vi "OFDM_TransimitPreparation.vi"(10 "IQ rate":dbl, 11 "array":cdb[](array[numeric])) -> (3 "output cluster":cluster{"t0":dbl, "dt":dbl, "Y":cdb[]})   [LabVIEW 2022 SP3]
uses:
  <vilib>/Analysis/baseanly.llb/Mean (DBL).vi
  <vilib>/Analysis/NI_AALBase.lvlib
panel:
  out "max index(es)":i32
  out "max value":dbl
  out "Average Power":dbl format="%0.6f"
  out "size(s)":i32
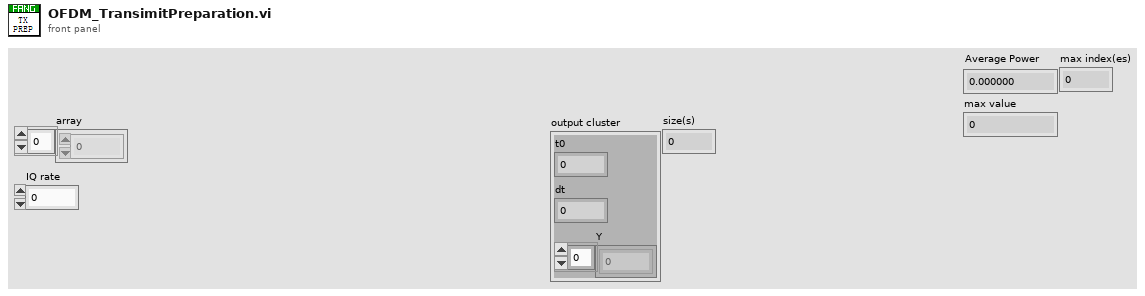
[diagram p1: front panel]
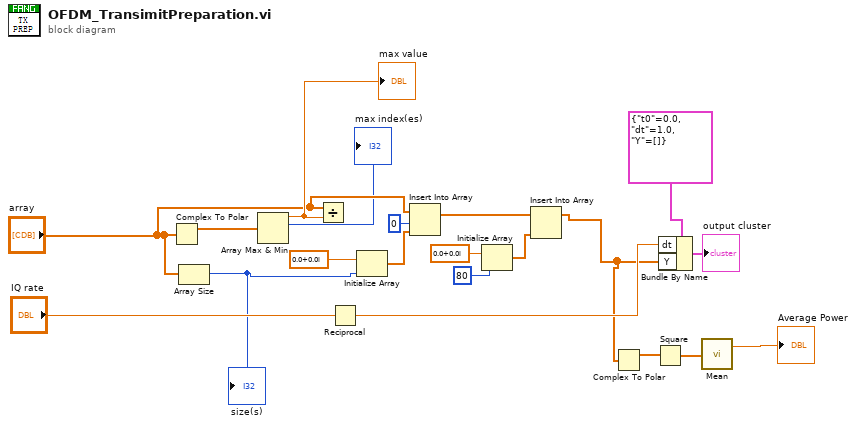
[diagram p0: block diagram]
diagram:
  n1 = Complex To Polar(r * e^(i*theta)="array") -> (r=w20:dbl[])  [unwired: 1 out]
  n2 = Array Size(array="array") -> (size(s)=w7:i32)
  "size(s)" <- w7
  n3 = Array Max & Min(array=w20) -> (max value=w19:dbl, max index (indices)=→"max index(es)":i32)  [unwired: 2 out]
  "max value" <- w19
  n4 = Divide(x="array", y=w19) -> ()  [unwired: 1 out]
  n5 = Reciprocal(x="IQ rate") -> (1/x=w9:dbl)
  n6 = Initialize Array(cdb 0.0+0.0i ("element"), w7) -> (w15:cdb[])
  n7 = Insert Into Array(array="array", index=0, new element=w15) -> (w16:cdb[])
  n8 = Initialize Array(cdb 0.0+0.0i ("element"), 80 ("dimension size")) -> (w14:cdb[])
  n9 = Insert Into Array(array=w16, new element=w14) -> (w3:cdb[])  [unwired: 1 in]
  n10 = Complex To Polar(r * e^(i*theta)=w3) -> (r=w6:dbl[])  [unwired: 1 out]
  n11 = Square(x=w6) -> (x^2=w5:dbl[])
  n12 = Bundle By Name(cluster=cluster{"t0":dbl, "dt":dbl, "Y":cdb[]} {"t0"=0.0, "dt"=1.0, "Y"=[]} ("data"), "dt"=w9, "Y"=w3) -> (→"output cluster":cluster{"t0":dbl, "dt":dbl, "Y":cdb[]})
  n13 = call-poly <vilib>:"Mean.vi"("X"=w5) -> ("mean"=→"Average Power":dbl)  [unwired: 1 out]
